vi "ExcelKit_SavePDFPrint.vi"() -> ()   [LabVIEW 2025]
panel:
  in  "ExcelKit.IExcelOperator":refnum<k7>
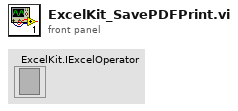
[diagram p1: front panel]
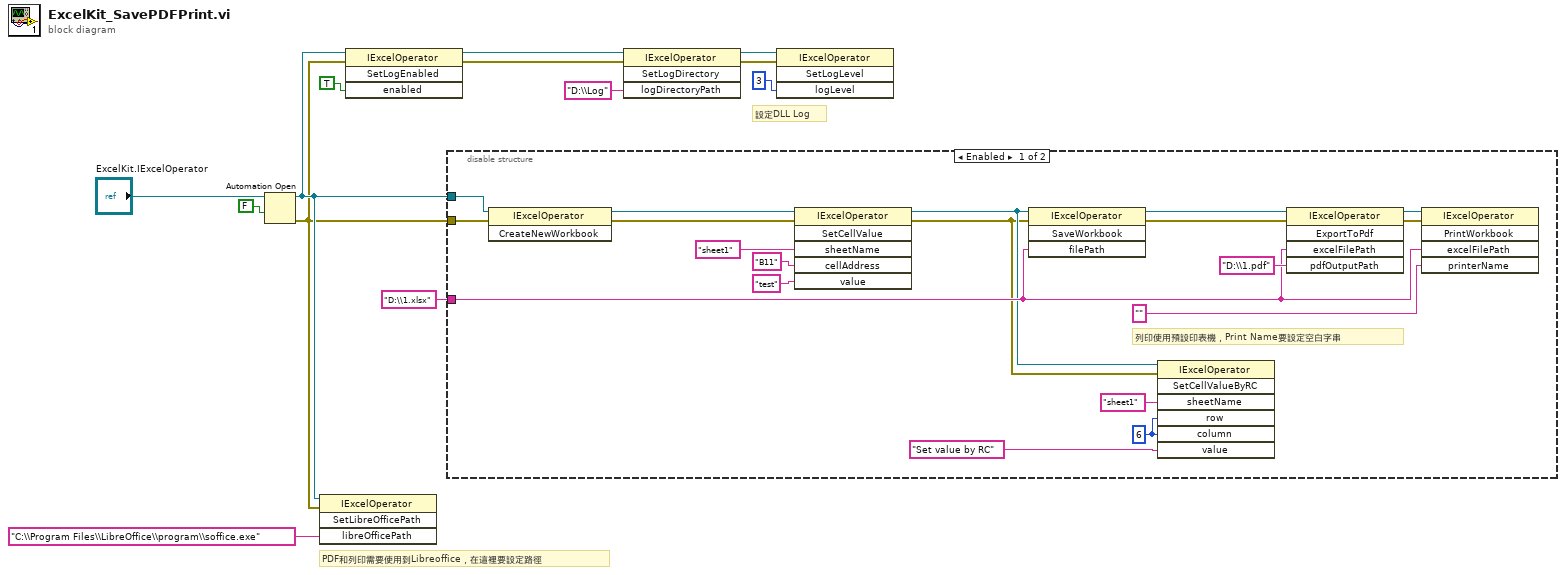
[diagram p0: block diagram]
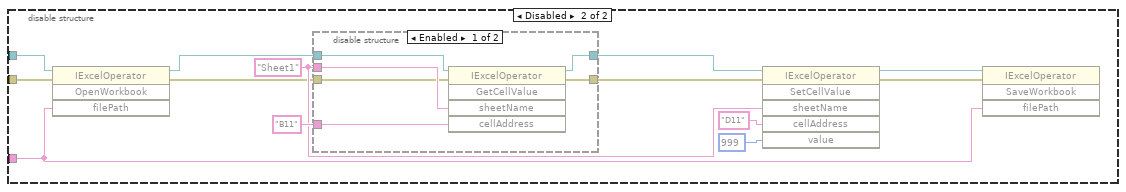
[diagram p2: hidden frame]
diagram:
  # "PDF和列印需要使用到Libreoffice，在這裡要設定路徑"
  # "設定DLL Log"
  n1 = Automation Open(Automation Refnum="ExcelKit.IExcelOperator", 9:FALSE ("open new instance (false)")) -> (Automation Refnum=w3:refnum<k7>, error out=w2:errorcluster)  [unwired: 2 in]
  n2 = invoke class="IExcelOperator" method="SetLibreOfficePath"(reference=w3, error in=w2, "libreOfficePath"="C:\\Program Files\\LibreOffice\\program\\soffice.exe") -> ()  [unwired: 1 in, 4 out]
  n3 = invoke class="IExcelOperator" method="SetLogEnabled"(reference=w3, error in=w2, "enabled"=TRUE) -> (reference out=w8:refnum<k7>, error out=w7:errorcluster)  [unwired: 1 in, 2 out]
  n4 = disable-structure shown="Enabled" {
    disable-tunnel: w3 -> [w32 w45]
    disable-tunnel: w2 -> [w29 w35]
    disable-tunnel: "D:\\1.xlsx" ("filePath") -> [w21 w37]
    frame Enabled {
      w15 = 6 ("row")
      # "列印使用預設印表機，Print Name要設定空白字串"
      n5 = invoke class="IExcelOperator" method="CreateNewWorkbook"(reference=w32, error in=w29) -> (reference out=w31:refnum<k7>, error out=w28:errorcluster)  [unwired: 1 in, 1 out]
      n6 = invoke class="IExcelOperator" method="SetCellValue"(reference=w31, error in=w28, "sheetName"="sheet1", "cellAddress"="B11", "value"="test" ("sheetName")) -> (reference out=w18:refnum<k7>, error out=w17:errorcluster)  [unwired: 1 in, 4 out]
      n7 = invoke class="IExcelOperator" method="SaveWorkbook"(reference=w18, error in=w17, "filePath"=w21) -> (reference out=w26:refnum<k7>, error out=w25:errorcluster)  [unwired: 1 in, 2 out]
      n8 = invoke class="IExcelOperator" method="SetCellValueByRC"(reference=w18, error in=w17, "sheetName"="sheet1", "row"=w15, "column"=w15, "value"="Set value by RC" ("sheetName")) -> ()  [unwired: 1 in, 7 out]
      n9 = invoke class="IExcelOperator" method="ExportToPdf"(reference=w26, error in=w25, "excelFilePath"=w21, "pdfOutputPath"="D:\\1.pdf") -> (reference out=w23:refnum<k7>, error out=w22:errorcluster)  [unwired: 1 in, 3 out]
      n10 = invoke class="IExcelOperator" method="PrintWorkbook"(reference=w23, error in=w22, "excelFilePath"=w21, "printerName"="") -> ()  [unwired: 1 in, 5 out]
    }
    frame Disabled {
      w41 = "Sheet1" ("sheetName")
      n11 = invoke class="IExcelOperator" method="OpenWorkbook"(reference=w45, error in=w35, "filePath"=w37) -> (reference out=w44:refnum<k7>, error out=w36:errorcluster)  [unwired: 1 in, 2 out]
      n12 = disable-structure shown="Enabled" {
        disable-tunnel: w44 -> [w52 w54]
        disable-tunnel: "B11" ("cellAddress") -> [w51 _]
        disable-tunnel: [w49 w54] -> w42
        disable-tunnel: w41 -> [w48 _]
        disable-tunnel: w36 -> [w47 w53]
        disable-tunnel: [w46 w53] -> w34
        frame Enabled {
          n13 = invoke class="IExcelOperator" method="GetCellValue"(reference=w52, error in=w47, "sheetName"=w48, "cellAddress"=w51) -> (reference out=w49:refnum<k7>, error out=w46:errorcluster, "GetCellValue"=w50:variant)  [unwired: 1 in, 2 out]
        }
        frame Disabled {
        }
      }
      n14 = invoke class="IExcelOperator" method="SetCellValue"(reference=w42, error in=w34, "sheetName"=w41, "cellAddress"="D11", "value"=999) -> (reference out=w38:refnum<k7>, error out=w33:errorcluster)  [unwired: 1 in, 4 out]
      n15 = invoke class="IExcelOperator" method="SaveWorkbook"(reference=w38, error in=w33, "filePath"=w37) -> ()  [unwired: 1 in, 4 out]
    }
  }
  n16 = invoke class="IExcelOperator" method="SetLogDirectory"(reference=w8, error in=w7, "logDirectoryPath"="D:\\Log") -> (reference out=w6:refnum<k7>, error out=w5:errorcluster)  [unwired: 1 in, 2 out]
  n17 = invoke class="IExcelOperator" method="SetLogLevel"(reference=w6, error in=w5, "logLevel"=3) -> ()  [unwired: 1 in, 4 out]
